vi "Start Sync.vi"(8 "error in (no error)":errorcluster, 11 "gRPC service in":refnum<class "OOBgRPCService.lvclass">) -> (0 "error out":errorcluster, 3 "gRPC service out":refnum<class "OOBgRPCService.lvclass">)   [LabVIEW 2025, in "OOB gRPC Server.lvlib" / "OOBgRPCService.lvclass"]
uses:
  OOBgRPCService.lvclass
  OOBgRPCService.lvclass/OOBgRPCService.ctl
  OOB Data Transfer/OOB Data Transfer.lvlib
  RPC Messages/hwval_GenericResponse.ctl
  OOB gRPC Server.lvlib
  RPC Messages/hwval_StatusResponse.ctl
  CAN-LIN Raw Bus Capture.lvclass
  Dequeue Frame.vi
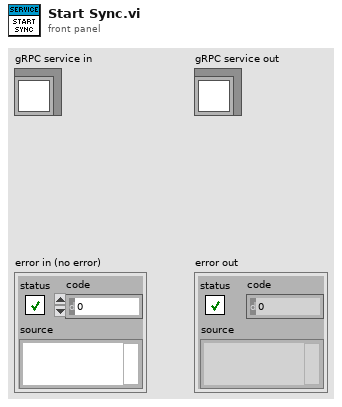
[diagram p1: front panel]
types:
  T1 = typedef "OOB gRPC Server.lvlib/hwval_GenericResponse.ctl" = cluster{"Payload":u8[]}
  T2 = typedef "OOB gRPC Server.lvlib/hwval_StatusResponse.ctl" = cluster{"Status":bool, "Code":i32, "Message":string}
  T3 = typedef "OOB gRPC Server.lvlib/OOBgRPCService.lvclass/Server Internal UEs.ctl" = cluster{"OOBgRPCService Generic Internal UE":refnum<user-event>, "OOBgRPCService PauseResume Internal UE":refnum<user-event>, "OOBgRPCService Export Internal UE":refnum<user-event>}
  T4 = typedef "OOB gRPC Server.lvlib/OOBgRPCService.lvclass/Server gRPC UEs.ctl" = cluster{"OOBgRPCService Generic gRPC UE":refnum<user-event>, "OOBgRPCService PauseResume gRPC UE":refnum<user-event>, "OOBgRPCService Export gRPC UE":refnum<user-event>}
  T5 = typedef "grpc-lvsupport-release.lvlib/grpcId.ctl" = u64
  T6 = typedef "OOB gRPC Server.lvlib/hwval_GenericRequest.ctl" = cluster{"Command":string, "Payload":u8[]}
  T7 = typedef "OOB Data Transfer.lvlib/OOB to Logic Data.ctl" = cluster{"PauseResume":bool, "Export":string}
  T8 = typedef "OOB gRPC Server.lvlib/hwval_BoolRequest.ctl" = cluster{"BooleanData":bool}
  T9 = typedef "OOB gRPC Server.lvlib/hwval_ExportRequest.ctl" = cluster{"FileType":string}
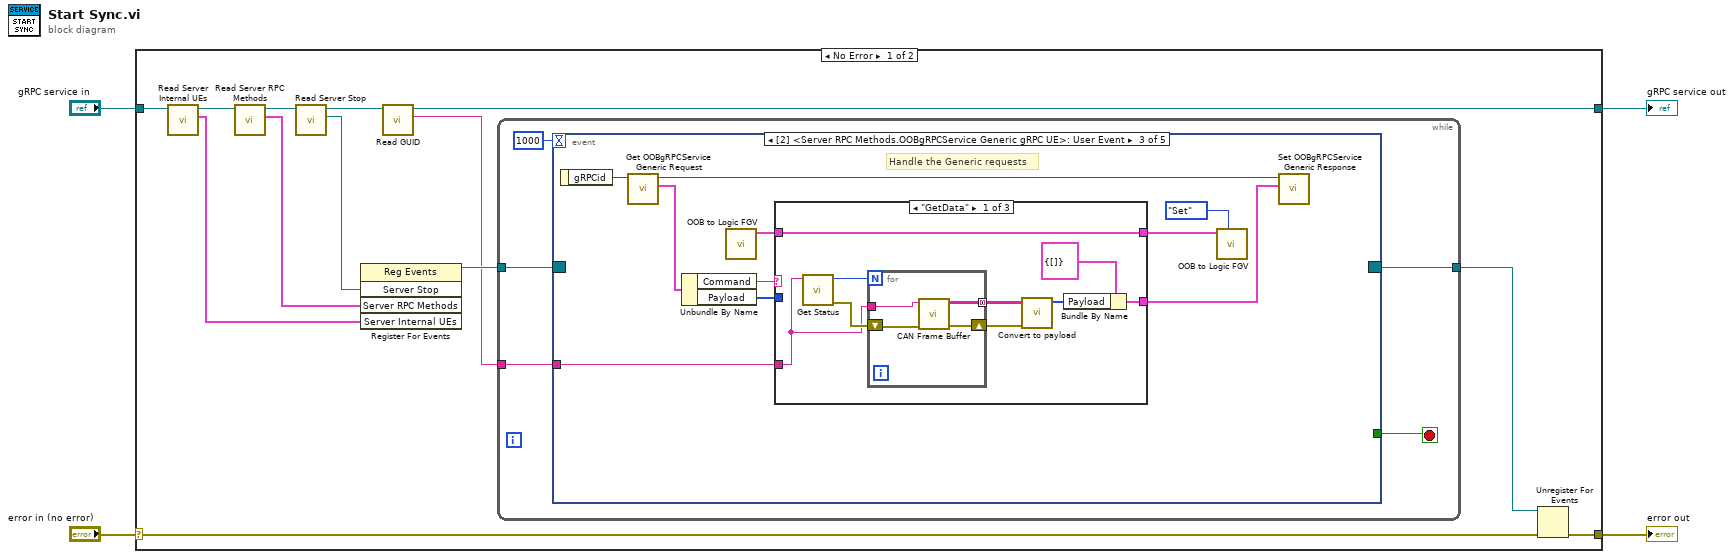
[diagram p0: block diagram]
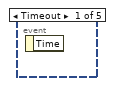
[diagram p2: hidden frame]
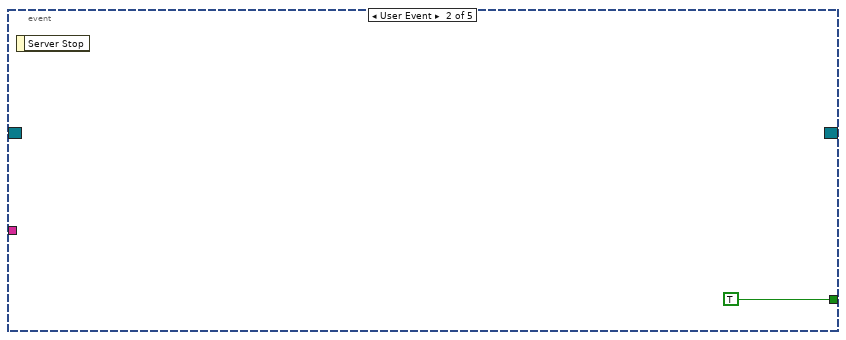
[diagram p3: hidden frame]
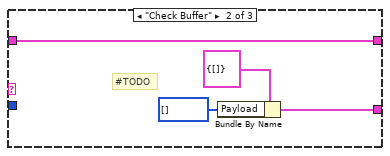
[diagram p4: hidden frame]
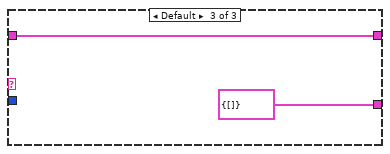
[diagram p5: hidden frame]
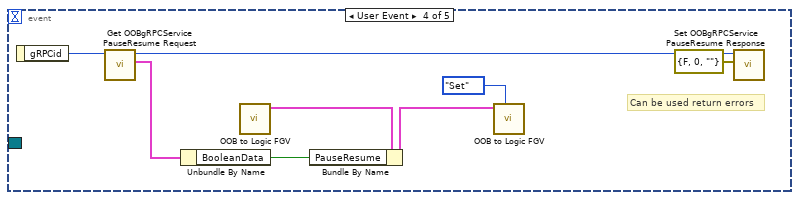
[diagram p6: hidden frame]
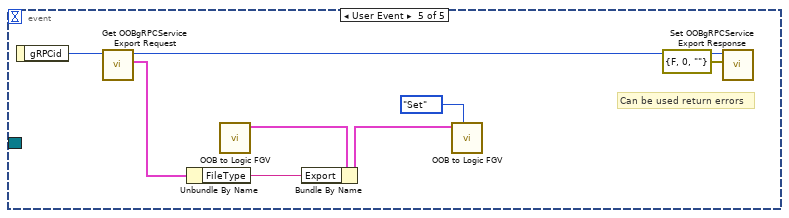
[diagram p7: hidden frame]
diagram:
  n1 = case shown="No Error" "error in (no error)" {
    selector: "error in (no error)" -> [w7 w70]
    tunnel: [w12 w70] -> w3
    tunnel: [w5 w69] -> w1
    tunnel: "gRPC service in" -> [w8 w69]
    frame No Error {
      n2 = call "Read Server Internal UEs.vi"("gRPC service in"=w8) -> ("Server Internal UEs"=w16:T3, "gRPC service out"=w17:refnum<class "OOBgRPCService.lvclass">)  [unwired: 8 in, 1 out]
      n3 = call "Read Server RPC Methods.vi"("gRPC service in"=w17) -> ("Server RPC Methods"=w11:T4, "gRPC service out"=w15:refnum<class "OOBgRPCService.lvclass">)  [unwired: 8 in, 1 out]
      n4 = call-dynamic "Read Server Stop.vi"("gRPC service in"=w15) -> ("Server Stop"=w10:refnum<user-event>, "gRPC service out"=w6:refnum<class "OOBgRPCService.lvclass">)  [unwired: 8 in, 1 out]
      n5 = register-events(w10, w11, w16) -> (reference out=w14:refnum<event-registration>)  [unwired: 2 in, 1 out]
      n6 = call "Read GUID.vi"("OOBgRPCService in"=w6) -> ("GUID"=w9:string, "OOBgRPCService out"=w5:refnum<class "OOBgRPCService.lvclass">)  [unwired: 8 in, 1 out]
      n7 = while {
        tunnel: w14 -> [w22]
        tunnel: [w20] -> w13
        tunnel: w9 -> [w18]
        stop <- w21 stop-if-true
        n8 = event "RPC Methods Event Structure" shown="[2] <Server RPC Methods.OOBgRPCService Generic gRPC UE>: User Event" {
          selector: w22 -> [_ _ _ _ _]
          dyn-events: [_ _ _ _ _] -> w20
          timeout: 1000 -> [_ _ _ _ _]
          tunnel: [_ TRUE _ _ _] -> w21
          tunnel: w18 -> [_ _ w24 _ _]
          event Timeout {
            n9 = event-data() -> ()  [unwired: 1 in, 1 out]
          }
          event User Event {
            n10 = event-data() -> ()  [unwired: 1 in, 1 out]
          }
          event User Event {
            # "Handle the Generic requests"
            n11 = event-data() -> ("gRPCid"=w33:T5)  [unwired: 1 in]
            n12 = call "Get OOBgRPCService Generic Request.vi"("gRPCid"=w33) -> ("Message Data"=w31:T6, "gRPCid out"=w32:T5)  [unwired: 8 in, 1 out]
            n13 = Unbundle By Name(w31) -> ("Command"=w27:string, "Payload"=w26:u8[])
            n14 = call "OOB to Logic FGV.vi"() -> ("OOB to Logic Data out"=w29:T7)  [unwired: 10 in, 1 out]
            n15 = case shown="\"GetData\"" w27 {
              tunnel: w29 -> [w42 w50 w51]
              tunnel: [w42 w50 w51] -> w28
              tunnel: w26 -> [_ _ _]
              tunnel: [w38 w48 T1 {"Payload"=[]} ("Message Data")] -> w25
              tunnel: w24 -> [w34 _ _]
              frame "GetData" {
                n16 = call "Get Status.vi"("GUID"=w34) -> ("error out"=w37:errorcluster, "Messages"=w36:i32)  [unwired: 9 in]
                n17 = for {
                  N: w36 -> [_]
                  shift-right: [w46] -> w41
                  shift-left: w37 -> [w45]
                  tunnel: [w44] -> w35 mode=concatenating
                  tunnel: w34 -> [w43]
                  n18 = call-poly "CAN Frame Buffer.vi"("error in"=w45, "GUID"=w43) -> ("error out"=w46:errorcluster, "Data"=w44:string[][])  [unwired: 8 in]
                }
                n19 = call "Convert to payload.vi"("error in"=w41, "Data"=w35) -> ("U8 Array"=w39:u8[])  [unwired: 8 in, 1 out]
                n20 = Bundle By Name(cluster=T1 {"Payload"=[]} ("Message Data"), "Payload"=w39) -> (w38:T1)
              }
              frame "Check Buffer" {
                # "#TODO"
                n21 = Bundle By Name(cluster=T1 {"Payload"=[]} ("Message Data"), "Payload"=u8[] []) -> (w48:T1)
              }
              frame Default {
              }
            }
            n22 = call "OOB to Logic FGV.vi"("Op (Get)"=enum16{"Get", "Set"}."Set", "OOB to Logic Data in"=w28) -> ()  [unwired: 8 in, 2 out]
            n23 = call "Set OOBgRPCService Generic Response.vi"("Message Data"=w25, "gRPCid in"=w32) -> ()  [unwired: 9 in, 1 out]
          }
          event User Event {
            # "Can be used return errors"
            n24 = event-data() -> ("gRPCid"=w54:T5)  [unwired: 1 in]
            n25 = call "Get OOBgRPCService PauseResume Request.vi"("gRPCid"=w54) -> ("Message Data"=w56:T8, "gRPCid out"=w57:T5)  [unwired: 8 in, 1 out]
            n26 = Unbundle By Name(w56) -> ("BooleanData"=w55:bool)
            n27 = call "OOB to Logic FGV.vi"() -> ("OOB to Logic Data out"=w59:T7)  [unwired: 10 in, 1 out]
            n28 = Bundle By Name(cluster=w59, "PauseResume"=w55) -> (w58:T7)
            n29 = call "OOB to Logic FGV.vi"("Op (Get)"=enum16{"Get", "Set"}."Set", "OOB to Logic Data in"=w58) -> ()  [unwired: 8 in, 2 out]
            n30 = call "Set OOBgRPCService PauseResume Response.vi"("Message Data"=T2 {"Status"=FALSE, "Code"=0, "Message"=""}, "gRPCid in"=w57) -> ()  [unwired: 9 in, 1 out]
          }
          event User Event {
            # "Can be used return errors"
            n31 = event-data() -> ("gRPCid"=w62:T5)  [unwired: 1 in]
            n32 = call "Get OOBgRPCService Export Request.vi"("gRPCid"=w62) -> ("Message Data"=w64:T9, "gRPCid out"=w68:T5)  [unwired: 8 in, 1 out]
            n33 = Unbundle By Name(w64) -> ("FileType"=w63:string)
            n34 = call "OOB to Logic FGV.vi"() -> ("OOB to Logic Data out"=w66:T7)  [unwired: 10 in, 1 out]
            n35 = Bundle By Name(cluster=w66, "Export"=w63) -> (w65:T7)
            n36 = call "OOB to Logic FGV.vi"("Op (Get)"=enum16{"Get", "Set"}."Set", "OOB to Logic Data in"=w65) -> ()  [unwired: 8 in, 2 out]
            n37 = call "Set OOBgRPCService Export Response.vi"("Message Data"=T2 {"Status"=FALSE, "Code"=0, "Message"=""}, "gRPCid in"=w68) -> ()  [unwired: 9 in, 1 out]
          }
        }
      }
      n38 = Unregister For Events(event registration refnum=w13, error in=w7) -> (error out=w12:errorcluster)
    }
    frame Error {
    }
  }
  "error out" <- w3
  "gRPC service out" <- w1
